vi "WLAN_FrameAnalysisV2.vi"(8 "error in (no error)":errorcluster, 10 "Modulation parameter LP":T1, 11 "input cluster":cluster{"t0":dbl, "dt":dbl, "Y":cdb[]}) -> (0 "error out":errorcluster, 1 "Constellation":cdb[](graph), 2 "Modulation parameter":T1, 3 "output bits":i8[](array[numeric]), 4 "Frequency offset":dbl, 5 "SIG valid?":bool, 6 "outputbitsHP":i8[](array[numeric]))   [LabVIEW 2022 SP3]
panel:
  out "subarray":cdb[](array[numeric])
  out "size(s) 6":i32
  out "size(s) 5":i32
  out "size(s) 4":i32
  out "x+y":dbl
  out "Frequency offset(LTF)":dbl
  out "Frequency offset corrected signal 2":cluster{"t0":dbl, "dt":dbl, "Y":dbl[]}(graph)
  out "size(s) 3":i32
  out "size(s) 2":i32
  out "size(s)":i32
  out "Symbol numbers":i32
  out "encoded bit numbers":u32
  out "original bit numbers":u32
  out "Channel Esitimate":dbl[](graph)
  out "Frequency offset corrected signal":cluster{"t0":dbl, "dt":dbl, "Y":dbl[]}(graph)
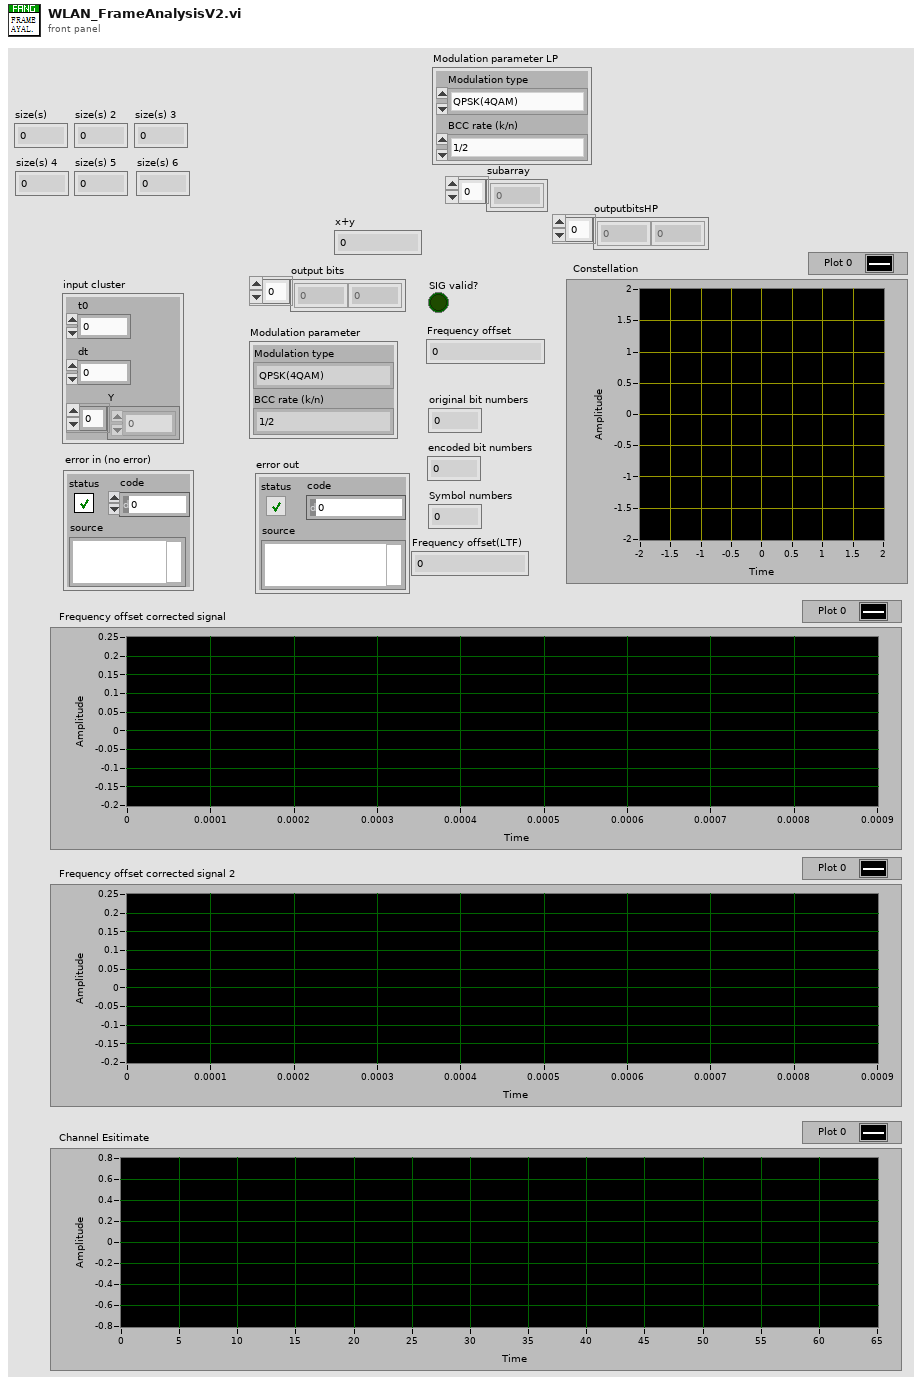
[diagram p1: front panel]
types:
  T1 = cluster{"Modulation type":enum16{"QPSK(4QAM)", "64QAM", "16QAM", "BPSK"}, "BCC rate (k/n)":enum16{"1/2", "2/3", "3/4"}}
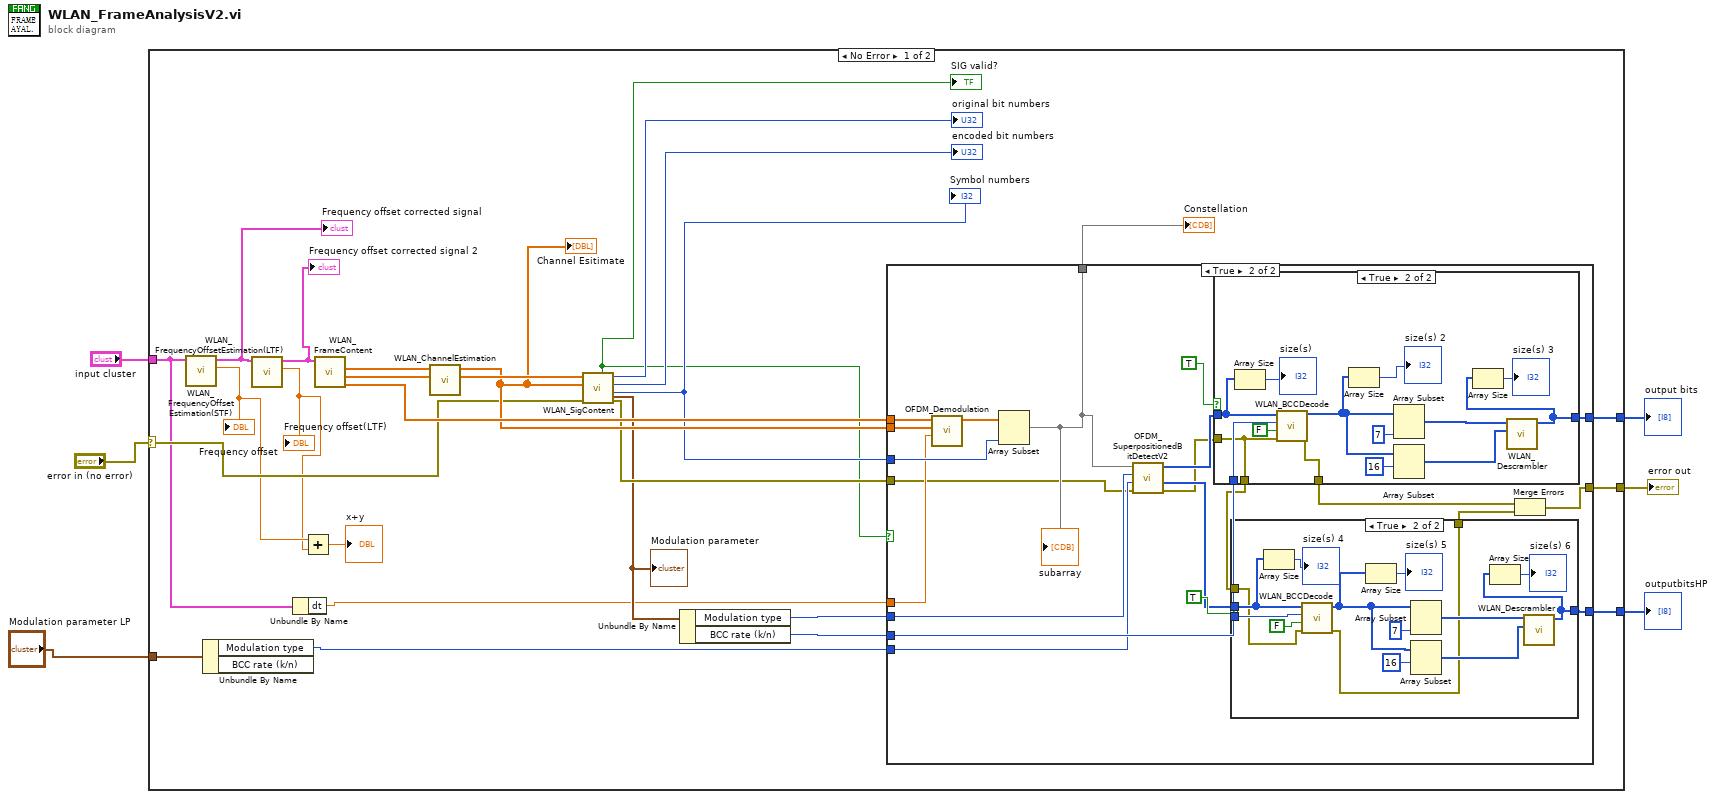
[diagram p0: block diagram]
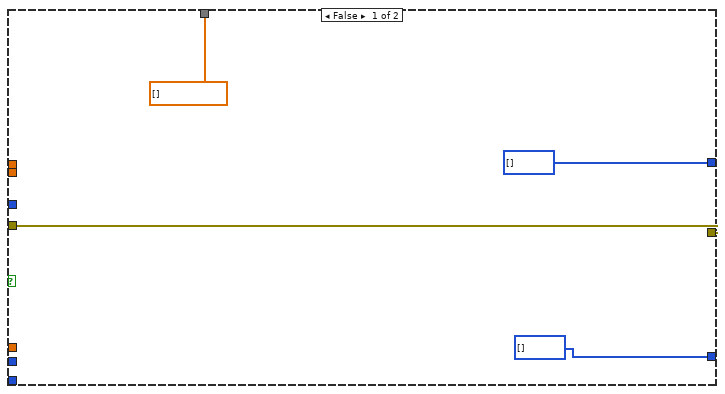
[diagram p2: hidden frame]
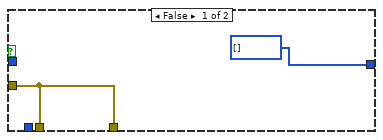
[diagram p3: hidden frame]
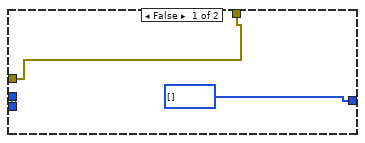
[diagram p4: hidden frame]
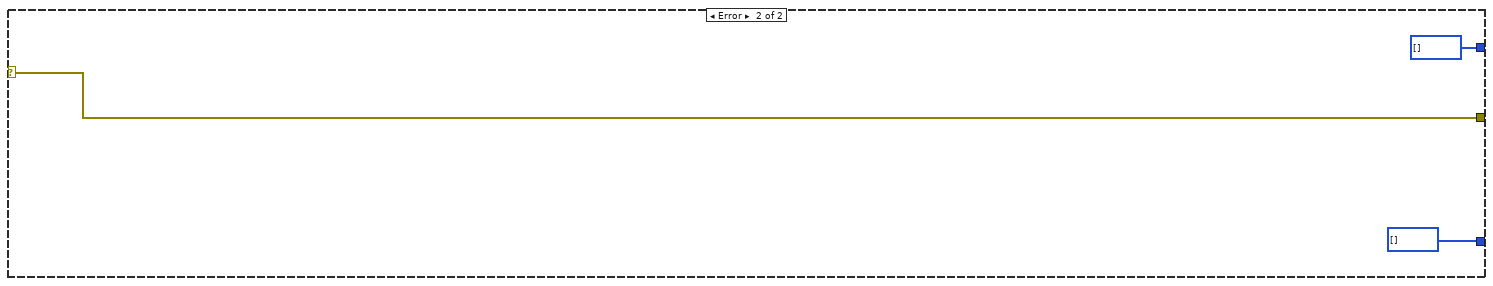
[diagram p5: hidden frame]
diagram:
  n1 = case shown="No Error" "error in (no error)" {
    selector: "error in (no error)" -> [w17 w91]
    tunnel: "input cluster" -> [w11 _]
    tunnel: [w24 w91] -> w5
    tunnel: [w23 i8[] [] ("scrambled bits")] -> w4
    tunnel: [w9 i8[] [] ("scrambled bits")] -> w2
    tunnel: "Modulation parameter LP" -> [w8 _]
    frame No Error {
      n2 = call "WLAN_FrequencyOffsetEstimation(STF).vi"("output cluster"=w11) -> ("Frequency offset(STF)"=w15:dbl, "output cluster 2"=w16:cluster{"t0":dbl, "dt":dbl, "Y":cdb[]})  [unwired: 8 in]
      "Frequency offset corrected signal" <- w16
      "Frequency offset" <- w15
      n3 = Unbundle By Name(w8) -> ("Modulation type"=w7:enum16{"QPSK(4QAM)", "64QAM", "16QAM", "BPSK"})  [unwired: 1 out]
      n4 = call "WLAN_FrequencyOffsetEstimation(LTF).vi"("input cluster"=w16) -> ("Frequency offset(LTF)"=w14:dbl, "output cluster"=w12:cluster{"t0":dbl, "dt":dbl, "Y":cdb[]})  [unwired: 9 in]
      "Frequency offset corrected signal 2" <- w12
      "Frequency offset(LTF)" <- w14
      n5 = Unbundle By Name(w11) -> ("dt"=w10:dbl)
      n6 = Add(x=w15, y=w14) -> (x+y=→"x+y":dbl)
      n7 = call "WLAN_FrameContent.vi"("Input cluster"=w12) -> ("DATA"=w32:cdb[], "SIG"=w30:cdb[], "LTF"=w31:cdb[])  [unwired: 7 in, 1 out]
      n8 = call "WLAN_ChannelEstimation.vi"("LTF"=w31) -> ("Frequency estimation"=w29:cdb[])  [unwired: 10 in]
      "Channel Esitimate" <- w29
      n9 = call "WLAN_SigContent.vi"("error in (no error)"=w17, "Frequency channel estimation"=w29, "SIG"=w30) -> ("error out"=w28:errorcluster, "Symbol numbers"=w25:i32, "encoded bit numbers"=→"encoded bit numbers":u32, "original bit numbers"=→"original bit numbers":u32, "Modulation parameter"=w22:T1, "SIG valid?"=w18:bool)  [unwired: 3 in]
      "Modulation parameter" <- w22
      "Symbol numbers" <- w25
      "SIG valid?" <- w18
      n10 = Unbundle By Name(w22) -> ("Modulation type"=w21:enum16{"QPSK(4QAM)", "64QAM", "16QAM", "BPSK"}, "BCC rate (k/n)"=w20:enum16{"1/2", "2/3", "3/4"})
      n11 = case shown="True" w18 {
        tunnel: w32 -> [_ w57]
        tunnel: [w36 w44] -> w24
        tunnel: w29 -> [_ w55]
        tunnel: w28 -> [w36 w40]
        tunnel: w25 -> [_ w54]
        tunnel: w21 -> [_ w42]
        tunnel: [i8[] [] ("scrambled bits") w53] -> w23
        tunnel: w20 -> [_ w51]
        tunnel: [cdb[] [] w43] -> w19
        tunnel: w10 -> [_ w52]
        tunnel: [i8[] [] ("scrambled bits") w50] -> w9
        tunnel: w7 -> [_ w41]
        frame False {
        }
        frame True {
          n12 = call "OFDM_Demodulation.vi"("sampling period"=w52, "Frequency channel estimation"=w55, "Input sequence"=w57) -> ("Output sequence"=w56:cdb[])  [unwired: 8 in]
          n13 = Array Subset(array=w56, length=w54) -> (w43:cdb[])  [unwired: 1 in]
          "subarray" <- w43
          n14 = call "OFDM_SuperpositionedBitDetectV2.vi"("error in (no error)"=w40, "Modulation type LP"=w41, "Modulation type"=w42, "Input symbols"=w43) -> ("error out"=w37:errorcluster, "OutputbitsHP"=w38:i8[], "OutputbitsLP"=w39:i8[])  [unwired: 5 in]
          n15 = case shown="True" TRUE ("need add zeros?") {
            tunnel: w37 -> [w58 w60]
            tunnel: [w58 w73] -> w46
            tunnel: w39 -> [_ w67]
            tunnel: [i8[] [] ("scrambled bits") w62] -> w53
            tunnel: w51 -> [_ w61]
            tunnel: [w58 w60] -> w47
            frame False {
            }
            frame True {
              n16 = Array Size(array=w67) -> (size(s)=→"size(s)":i32)
              n17 = call "WLAN_BCCDecode.vi"("error in (no error)"=w60, "need add zeros?"=FALSE, "BCC rate (k/n)"=w61, "input bit stream"=w67) -> ("error out"=w73:errorcluster, "output bit stream"=w64:i8[])  [unwired: 6 in]
              n18 = Array Size(array=w64) -> (size(s)=→"size(s) 2":i32)
              n19 = Array Subset(array=w64, length=7) -> (w69:i8[])  [unwired: 1 in]
              n20 = Array Subset(array=w64, index=16) -> (w70:i8[])  [unwired: 1 in]
              n21 = call "WLAN_Descrambler.vi"("scrambler initial bits"=w69, "data bits"=w70) -> ("scrambled bits"=w62:i8[])  [unwired: 7 in]
              n22 = Array Size(array=w62) -> (size(s)=→"size(s) 3":i32)
            }
          }
          n23 = case shown="True" TRUE ("need add zeros?") {
            tunnel: w51 -> [_ w88]
            tunnel: w38 -> [_ w87]
            tunnel: [i8[] [] ("scrambled bits") w76] -> w50
            tunnel: w47 -> [w74 w78]
            tunnel: [w74 w77] -> w45
            frame False {
            }
            frame True {
              n24 = Array Size(array=w87) -> (size(s)=→"size(s) 4":i32)
              n25 = call "WLAN_BCCDecode.vi"("error in (no error)"=w78, "need add zeros?"=FALSE, "BCC rate (k/n)"=w88, "input bit stream"=w87) -> ("error out"=w77:errorcluster, "output bit stream"=w84:i8[])  [unwired: 6 in]
              n26 = Array Size(array=w84) -> (size(s)=→"size(s) 5":i32)
              n27 = Array Subset(array=w84, length=7) -> (w80:i8[])  [unwired: 1 in]
              n28 = Array Subset(array=w84, index=16) -> (w81:i8[])  [unwired: 1 in]
              n29 = call "WLAN_Descrambler.vi"("scrambler initial bits"=w80, "data bits"=w81) -> ("scrambled bits"=w76:i8[])  [unwired: 7 in]
              n30 = Array Size(array=w76) -> (size(s)=→"size(s) 6":i32)
            }
          }
          n31 = Merge Errors(w46, w45) -> (w44:errorcluster)
        }
      }
      "Constellation" <- w19
    }
    frame Error {
    }
  }
  "error out" <- w5
  "output bits" <- w4
  "outputbitsHP" <- w2
